vi "Post-Install Custom Action.vi"(10 "Variant":variant) -> (0 "error out":errorcluster)   [LabVIEW 2017]
uses:
  <vilib>/Utility/traverseref.llb/TRef TravTarget.ctl
  <vilib>/Utility/traverseref.llb/VI Scripting - Traverse.lvlib
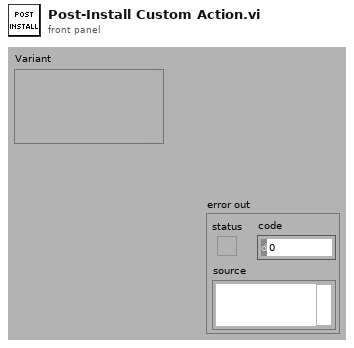
[diagram p1: front panel]
types:
  T1 = typedef "TRef TravTarget.ctl" = enum16{"FP", "BD", "Other"}
  T2 = enum32{"invalid VI type", "Standard VI", "Control VI", "Global VI", "Polymorphic VI", "Configuration VI", "SubSystem", "Facade VI", "Method VI", "Statechart Diagram VI"}
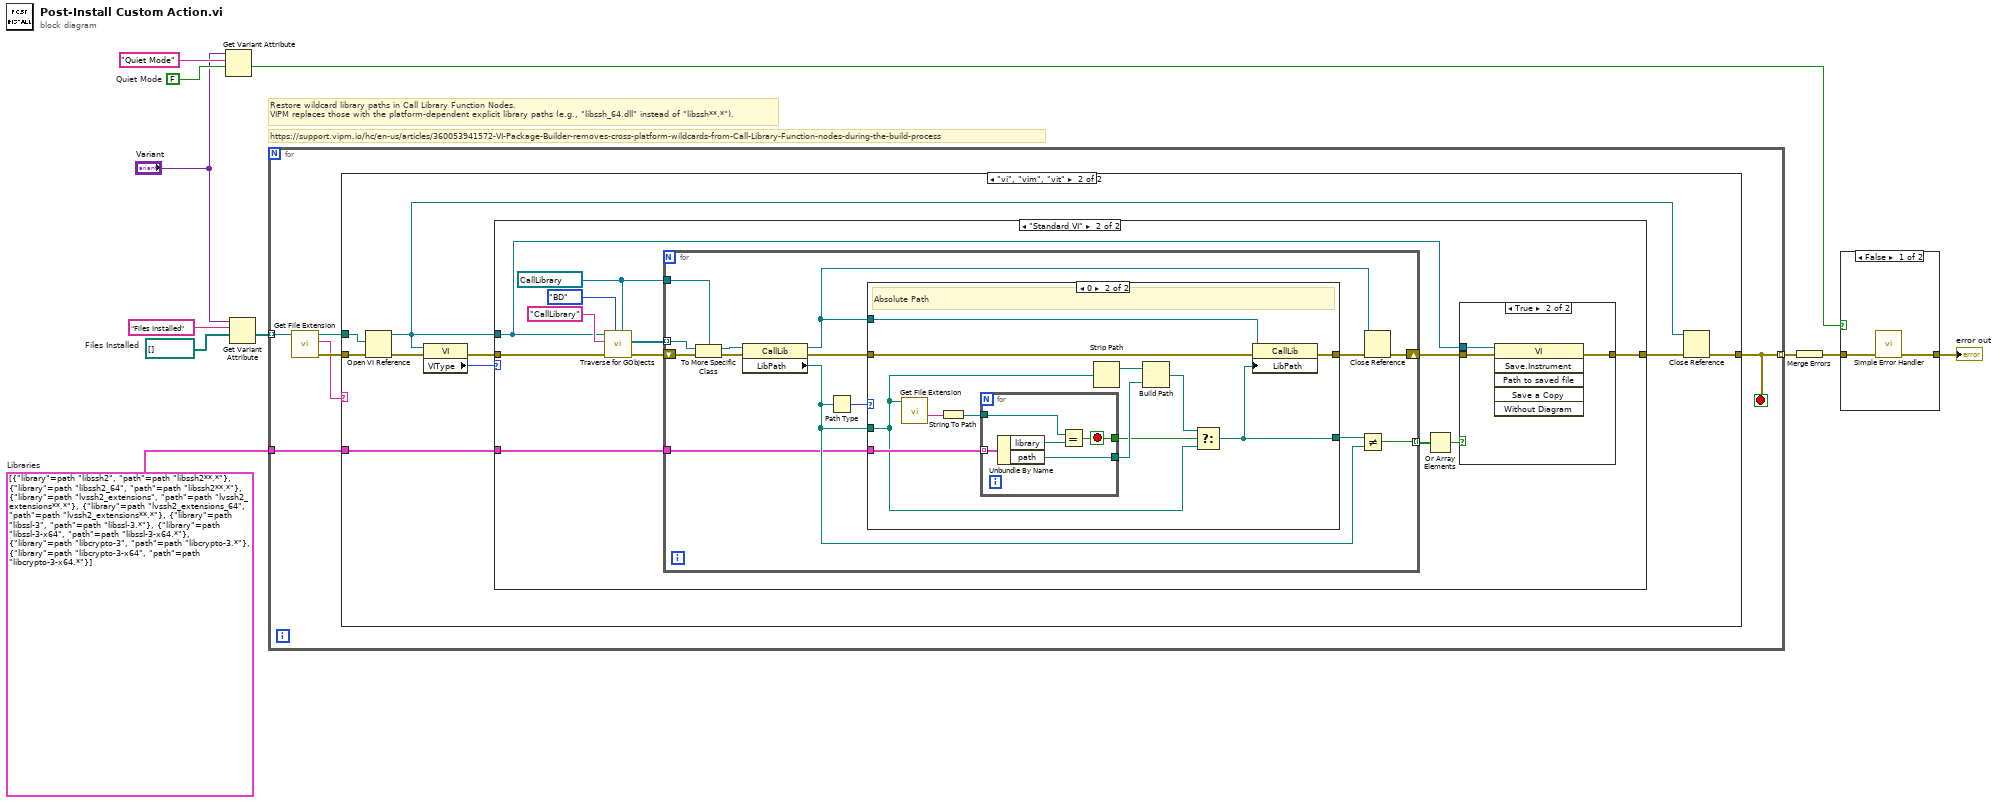
[diagram p0: block diagram]
diagram:
  w1 = cluster{"library":path, "path":path}[] [{"library"=path "libssh2", "path"=path "libssh2**.*"}, {"library"=path "libssh2_64", "path"=path "libssh2**.*"}, {"library"=path "lvssh2_extensions", "path"=path "lvssh2_extensions**.*"}, {"library"=path "lvssh2_extensions_64", "path"=path "lvssh2_extensions**.*"}, {"library"=path "libssl-3", "path"=path "libssl-3.*"}, {"library"=path "libssl-3-x64", "path"=path "libssl-3-x64.*"}, {"library"=path "libcrypto-3", "path"=path "libcrypto-3.*"}, {"library"=path "libcrypto-3-x64", "path"=path "libcrypto-3-x64.*"}]  # Libraries
  w6 = FALSE  # Quiet Mode
  w10 = path[] []  # Files Installed
  # "Restore wildcard library paths in Call Library Function Nodes.\nVIPM replaces those with the platform-dependent explicit library paths (e.g., \"libssh_64.dll\" instead of \"libssh**.*\")."
  # "https://support.vipm.io/hc/en-us/articles/360053941572-VI-Package-Builder-removes-cross-platform-wildcards-from-Call-Library-Function-nodes-during-the-build-process"
  n1 = Get Variant Attribute(Variant="Variant", name="Quiet Mode", default value (empty Variant)=w6) -> (value=w2:bool)  [unwired: 1 in, 3 out]
  n2 = Get Variant Attribute(Variant="Variant", name="Files Installed", default value (empty Variant)=w10) -> (value=w9:path[])  [unwired: 1 in, 3 out]
  n3 = for {
    tunnel: w9 -> [w17] mode=indexing
    tunnel: [w13] -> w8 mode=indexing
    tunnel: w1 -> [w12]
    stop <- w13 stop-if-true
    n4 = call <vilib>:"Get File Extension.vi"("file"=w17) -> ("error out"=w15:errorcluster, "lowercase file extension"=w14:string, "dup file"=w16:path)  [unwired: 6 in, 2 out]
    n5 = case shown="\"vi\", \"vim\", \"vit\"" w14 {
      tunnel: w16 -> [_ w27]
      tunnel: [w18 w25] -> w13
      tunnel: w15 -> [w18 w24]
      tunnel: w12 -> [_ w19]
      frame Default {
      }
      frame "vi", "vim", "vit" {
        n6 = Open VI Reference(vi path=w27, error in (no error)=w24) -> (vi reference=w21:refnum<vi>, error out=w23:errorcluster)  [unwired: 4 in]
        n7 = property class="VI"(reference=w21, error in=w23) -> (error out=w22:errorcluster, "VIType"=w20:T2)  [unwired: 1 out]
        n8 = case shown="\"Standard VI\"" w20 {
          tunnel: [w28 w32] -> w26
          tunnel: w22 -> [w28 w31]
          tunnel: w21 -> [_ w30]
          tunnel: w19 -> [_ w29]
          frame Default {
            # "Polimorphic VIs, etc."
          }
          frame "Standard VI" {
            w36 = refnum<vi> refnum ("Other Refnum")
            n9 = call <vilib>:"Traverse for GObjects.vi"("Other Refnum"=w36, "Traverse Target"=TRef_TravTarget."BD", "error in (no error)"=w31, "Class Name"="CallLibrary", "VI Refnum"=w30) -> ("error out"=w37:errorcluster, "References"=w38:refnum<vi>[])  [unwired: 3 in, 2 out]
            n10 = for {
              tunnel: w38 -> [w56] mode=indexing
              shift-right: [w50] -> w33
              shift-left: w37 -> [w58]
              tunnel: w36 -> [w57]
              tunnel: [w46] -> w35 mode=indexing
              tunnel: w29 -> [w45]
              n11 = To More Specific Class(target class=w57, reference=w56, error in=w58) -> (specific class reference=w54:refnum<vi>, error out=w55:errorcluster)
              n12 = property class="CallLib"(reference=w54, error in=w55) -> (reference out=w49:refnum<vi>, error out=w51:errorcluster, "LibPath"=w47:path)
              n13 = Path Type(1:w47) -> (0:w53:i16)
              n14 = case shown="0" w53 {
                tunnel: [w60 w72] -> w52
                tunnel: w51 -> [w60 w64]
                tunnel: w47 -> [w59 w61]
                tunnel: w49 -> [_ w71]
                tunnel: [w59 w62] -> w48
                tunnel: w45 -> [_ w69]
                frame Default {
                  # "kernel32.dll, etc."
                  # "Relative / <Not A Path>"
                }
                frame 0 {
                  # "Absolute Path"
                  n15 = call <vilib>:"Get File Extension.vi"("file"=w61) -> ("filename without extension"=w70:string)  [unwired: 6 in, 4 out]
                  n16 = String To Path(string=w70) -> (path=w68:path)
                  n17 = for {
                    tunnel: w69 -> [w77] mode=indexing
                    tunnel: w68 -> [w75]
                    tunnel: [w74] -> w67
                    tunnel: [w73] -> w66
                    stop <- w73 stop-if-true
                    n18 = Unbundle By Name(w77) -> ("library"=w76:path, "path"=w74:path)
                    n19 = Equal?(x=w75, y=w76) -> (x = y?=w73:bool)
                  }
                  n20 = Strip Path(path=w61) -> (stripped path=w65:path)  [unwired: 1 out]
                  n21 = Build Path(base path=w65, name or relative path=w67) -> (appended path=w63:path)
                  n22 = Select(t=w63, s=w66, f=w61) -> (s? t:f=w62:path)
                  n23 = property class="CallLib"(reference=w71, error in=w64, "LibPath"=w62) -> (error out=w72:errorcluster)  [unwired: 1 out]
                }
              }
              n24 = Not Equal?(x=w48, y=w47) -> (x != y?=w46:bool)
              n25 = Close Reference(reference=w49, error in (no error)=w52) -> (error out=w50:errorcluster)
            }
            n26 = Or Array Elements(Boolean array=w35) -> (logical OR=w34:bool)
            n27 = case shown="True" w34 {
              tunnel: w30 -> [_ w44]
              tunnel: w33 -> [w41 w43]
              tunnel: [w41 w42] -> w32
              frame False {
              }
              frame True {
                n28 = invoke class="VI" method="Save.Instrument"(reference=w44, error in=w43) -> (error out=w42:errorcluster)  [unwired: 4 in, 5 out]
              }
            }
          }
        }
        n29 = Close Reference(reference=w21, error in (no error)=w26) -> (error out=w25:errorcluster)
      }
    }
  }
  n30 = Merge Errors(w8) -> (w3:errorcluster)
  n31 = case shown="False" w2 {
    tunnel: [w78 w80] -> w4
    tunnel: w3 -> [w79 w80]
    frame False {
      n32 = call <vilib>:"Simple Error Handler.vi"("error in (no error)"=w79) -> ("error out"=w78:errorcluster)  [unwired: 4 in, 4 out]
    }
    frame True {
    }
  }
  "error out" <- w4
